vi "WaitForCtrlRef.vi"(0 "VI Reference In":refnum<vi>, 5 "Control Path":string, 7 "Timeout(ms)":u32=10000, 11 "Error In":errorcluster) -> (4 "VI Reference Out":refnum<vi>, 15 "Error Out":errorcluster)   [LabVIEW 2019, in "Drona.lvlib"]
doc: "This VI waits until the control reference will be available or until timeout"
uses:
  Drona.lvlib
  APIs/Get/GetControlRef/GetControlRefByPath.vi
  APIs/Get/GetControlRef/GetControlRef.lvlib
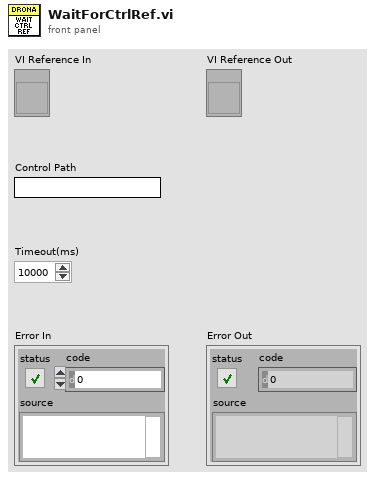
[diagram p1: front panel]
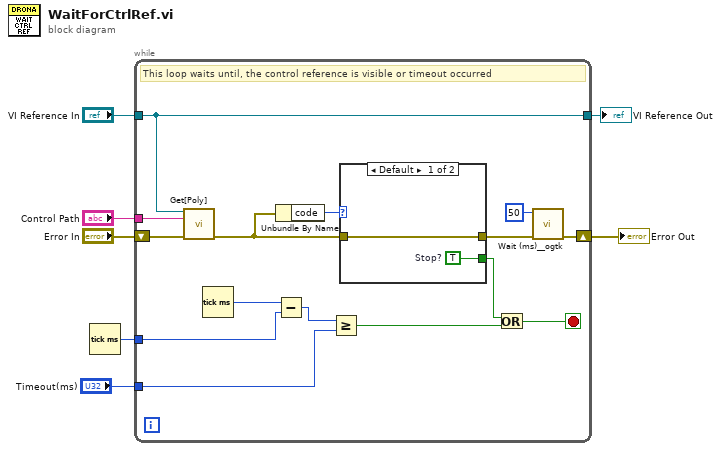
[diagram p0: block diagram]
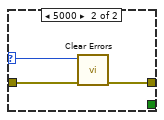
[diagram p2: hidden frame]
diagram:
  n1 = Tick Count (ms)() -> (millisecond timer value=w4:u32)
  n2 = while {
    tunnel: "VI Reference In" -> [w14]
    tunnel: "Control Path" -> [w21]
    tunnel: w4 -> [w20]
    tunnel: "Timeout(ms)" -> [w19]
    shift-right: [w9] -> w2
    shift-left: "Error In" -> [w22]
    tunnel: [w14] -> w1
    stop <- w11 stop-if-true
    # "This loop waits until, the control reference is visible or timeout occurred"
    n3 = call-poly "Get[Poly].vi"("VI Reference In"=w14, "Control Path"=w21, "error In"=w22) -> ("error out"=w16:errorcluster)  [unwired: 10 in, 2 out]
    n4 = Tick Count (ms)() -> (millisecond timer value=w18:u32)
    n5 = Unbundle By Name(w16) -> ("code"=w15:i32)
    n6 = Subtract(x=w18, y=w20) -> (x-y=w17:u32)
    n7 = Greater Or Equal?(x=w17, y=w19) -> (x >= y?=w13:bool)
    n8 = case shown="Default" w15 {
      selector: w15 -> [_ w25]
      tunnel: w16 -> [w24 w27]
      tunnel: [w24 w26] -> w10
      tunnel: [w23 _] -> w12
      frame Default {
        w23 = TRUE  # Stop?
      }
      frame 5000 {
        n9 = call <vilib>:"Clear Errors.vi"("error in (no error)"=w27, "specific error code to clear (0: all)"=w25) -> ("error out"=w26:errorcluster)  [unwired: 4 in, 1 out]
      }
    }
    n10 = Or(x=w12, y=w13) -> (x .or. y?=w11:bool)
    n11 = call <userlib>:"Wait (ms)__ogtk.vi"("error in (no error)"=w10, "milliseconds to wait"=u32 50) -> ("error out"=w9:errorcluster)  [unwired: 8 in, 1 out]
  }
  "Error Out" <- w2
  "VI Reference Out" <- w1
